vi "List Available Tags.vi"(8 "error in (no error)":errorcluster, 10 "engine":refnum<data-value>, 11 "E2E editor node in":refnum<data-value>) -> (0 "error out":errorcluster, 1 "Available Tags":refnum<class "tag descriptor.lvclass">[](array[class]), 2 "engine out":refnum<data-value>, 3 "E2E editor node out":refnum<data-value>)   [LabVIEW 2015, in "E2E Tag Exchange editor node.lvclass"]
uses:
  E2E Tag Exchange editor node.lvclass
  <vilib>/NI/DCAF/Tag Editor Core/Configuration Editor/Classes/Engine Parent/Engine Parent Editor Node.lvclass
  <vilib>/NI/Tag Bus/tag/tag descriptor.lvclass
  E2E Tag Exchange editor node.lvclass/E2E Tag Exchange editor node.ctl
  <vilib>/NI/Configuration Framework/serializable configuration/NISE_CEF_serializable configuration.lvclass/NISE_CEF_serializable configuration.ctl
  <vilib>/NI/Module Execution Interface/Engine Configuration/engine configuration.lvclass/engine configuration.ctl
  <vilib>/NI/Tag Bus/tag/tag descriptor.lvclass/tag descriptor.ctl
  <vilib>/Utility/LVClass/Get LV Class Name.vi
  <vilib>/NI/Configuration Framework/error generator/NISE_error generator.vi
  <vilib>/NI/Module Execution Interface/Engine Configuration/engine configuration.lvclass
  module/configuration/E2E Tag Exchange configuration.lvclass
  <vilib>/NI/Configuration Framework/serializable configuration/NISE_CEF_serializable configuration.lvclass
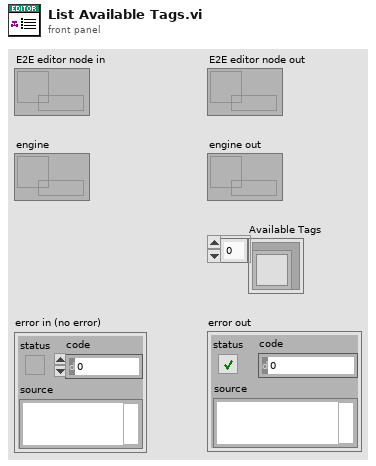
[diagram p1: front panel]
types:
  T1 = typedef "tag bus.lvlib/tag descriptor.lvclass/Data Type.ctl" = enum16{"Double", "Single", "I64", "I32", "I16", "I8", "U64", "U32", "U16", "U8", "Boolean", "String", "Array of Double", "Array of Single", "Array of I64", "Array of I32", "Array of I16", "Array of I8", "Array of U64", "Array of U32", "Array of U16", "Array of U8", "Array of Boolean", "Array of String"}
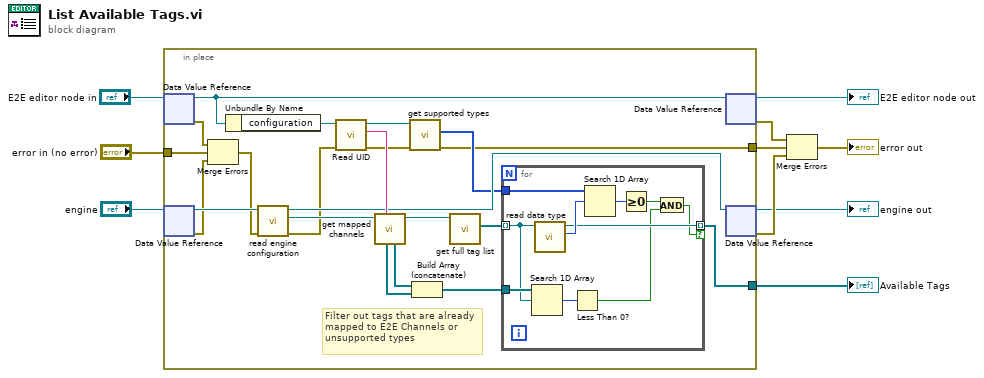
[diagram p0: block diagram]
diagram:
  n1 = in-place {
    in-place-border: "error in (no error)" -> [w18]
    in-place-border: [w20] -> w3
    in-place-border: [w11] -> w6
    # "Filter out tags that are already\nmapped to E2E Channels or \nunsupported types"
    n2 = in-place-dvr #1("E2E editor node in") -> (w22:refnum<class "E2E Tag Exchange editor node.lvclass">, w19:errorcluster)
    n3 = in-place-dvr #2("engine") -> (w31:refnum<class "Engine Parent Editor Node.lvclass">, w17:errorcluster)
    n4 = Merge Errors(w19, w18, w17) -> (w16:errorcluster)
    n5 = Unbundle By Name(w22) -> ("configuration"=w30:refnum<class "E2E Tag Exchange configuration.lvclass">)
    n6 = call <vilib>:"read engine configuration.vi"("error in"=w16, "Engine Parent Editor Node in"=w31) -> ("error out"=w15:errorcluster, "engine configuration"=w29:refnum<class "engine configuration.lvclass">, "Engine Parent Editor Node out"=w21:refnum<class "Engine Parent Editor Node.lvclass">)  [unwired: 7 in]
    n7 = call <vilib>:"Read UID.vi"("error in"=w15, "configuration in"=w30) -> ("error out"=w14:errorcluster, "instance id"=w28:string, "configuration out"=w13:refnum<class "E2E Tag Exchange configuration.lvclass">)  [unwired: 7 in]
    n8 = call-dynamic "get mapped channels.vi"("owner"=w28, "engine configuration in"=w29) -> ("engine configuration out"=w27:refnum<class "engine configuration.lvclass">, "paired read tag"=w25:refnum<class "tag descriptor.lvclass">[], "paired write tag"=w24:refnum<class "tag descriptor.lvclass">[])  [unwired: 5 in, 2 out]
    n9 = call-dynamic "get supported types.vi"("error in"=w14, "E2E Tag Exchange configuration in"=w13) -> ("error out"=w11:errorcluster, "supported types"=w12:T1[])  [unwired: 7 in, 1 out]
    n10 = Build Array (concatenate)(w25, w24) -> (w23:refnum<class "tag descriptor.lvclass">[])
    n11 = call <vilib>:"get full tag list.vi"("engine configuration in"=w27) -> ("tag list"=w26:refnum<class "tag descriptor.lvclass">[])  [unwired: 9 in, 1 out]
    n12 = for {
      tunnel: w26 -> [w39] mode=indexing
      tunnel: w23 -> [w41]
      tunnel: [w35] -> w20 mode=indexing if=w32
      tunnel: w12 -> [w38]
      n13 = Search 1D Array(1D array=w41, element=w39) -> (index of element=w40:i32)  [unwired: 1 in]
      n14 = call <vilib>:"read data type.vi"("system tag in"=w39) -> ("data type"=w37:T1, "system tag out"=w35:refnum<class "tag descriptor.lvclass">)  [unwired: 8 in, 1 out]
      n15 = Less Than 0?(x=w40) -> (x < 0?=w33:bool)
      n16 = Search 1D Array(1D array=w38, element=w37) -> (index of element=w36:i32)  [unwired: 1 in]
      n17 = Greater Or Equal To 0?(x=w36) -> (x >= 0?=w34:bool)
      n18 = And(x=w34, y=w33) -> (x .and. y?=w32:bool)
    }
    n19 = in-place-dvr #1(w22) -> (→"E2E editor node out":refnum<data-value>, w7:errorcluster)
    n20 = in-place-dvr #2(w21) -> (→"engine out":refnum<data-value>, w5:errorcluster)
  }
  "Available Tags" <- w3
  n21 = Merge Errors(w7, w6, w5) -> (→"error out":errorcluster)
